vi "read-json-testing.vi"() -> ()   [LabVIEW 2019]
uses:
  <vilib>/Rock Robotics/WPI/ThirdParty/MJansen/PathPlanner/TypeDef/PathPlannerPath.ctl
  <vilib>/Rock Robotics/WPI/ThirdParty/MJansen/PathPlanner/TypeDef/PathPlannerRotationTarget.ctl
  <vilib>/Rock Robotics/WPI/ThirdParty/JAS_Junk/TrajLib/TypeDef/ROTATION2D.ctl
  <vilib>/Rock Robotics/WPI/ThirdParty/MJansen/PathPlanner/TypeDef/PathPlannerConstraintsZone.ctl
  <vilib>/Rock Robotics/WPI/ThirdParty/MJansen/PathPlanner/TypeDef/PathPlannerPathConstraints.ctl
  <vilib>/Rock Robotics/WPI/ThirdParty/MJansen/PathPlanner/TypeDef/PathPlannerEventMarker.ctl
  <vilib>/Rock Robotics/WPI/ThirdParty/MJansen/PathPlanner/TypeDef/PathPlannerCommandUtil.ctl
  <vilib>/Rock Robotics/WPI/ThirdParty/MJansen/PathPlanner/ENum/PathPlanner_CommandUtilType_ENUM.ctl
  <vilib>/Rock Robotics/WPI/ThirdParty/MJansen/PathPlanner/TypeDef/PathPlannerGoalEndState.ctl
  <vilib>/Rock Robotics/WPI/ThirdParty/MJansen/PathPlanner/TypeDef/PathPlannerPathPoint.ctl
  <vilib>/Rock Robotics/WPI/ThirdParty/JAS_Junk/TrajLib/TypeDef/TRANSLATION2D.ctl
  <vilib>/Rock Robotics/WPI/ThirdParty/MJansen/PathPlanner/TypeDef/PathPlannerWaypoint.ctl
  <vilib>/Rock Robotics/WPI/ThirdParty/MJansen/PathPlanner/TypeDef/PathPlannerPointTowardsZone.ctl
  <vilib>/Rock Robotics/WPI/ThirdParty/MJansen/PathPlanner/TypeDef/PathPlannerIdealStartingState.ctl
  <vilib>/Rock Robotics/WPI/ThirdParty/MJansen/PathPlanner/TypeDef/PathPlannerTrajectory.ctl
  <vilib>/Rock Robotics/WPI/ThirdParty/MJansen/PathPlanner/TypeDef/PathPlannerTrajectoryState.ctl
  <vilib>/Rock Robotics/WPI/ThirdParty/JAS_Junk/TrajLib/TypeDef/CHASSIS_SPEEDS.ctl
  <vilib>/Rock Robotics/WPI/ThirdParty/MJansen/PathPlanner/VI/PathPlanner_EventMarker_New.vi
  <vilib>/Rock Robotics/WPI/ThirdParty/MJansen/PathPlanner/VI/PathPlanner_CommandUtil_TypeFromString.vi
  <vilib>/Rock Robotics/WPI/ThirdParty/MJansen/PathPlanner/VI/PathPlanner_EventMarker_FromJSON_Data.vi
  <vilib>/Rock Robotics/WPI/ThirdParty/MJansen/PathPlanner/PathPlanner24.lvlib
  <vilib>/Rock Robotics/WPI/ThirdParty/JAS_Junk/TrajLib/Trajectory_Library.lvlib
panel:
  out "Exists":bool
  out "EventMarkers":T1[](array[typedef])
  in  "StartingSpeeds":T4 {"vOmega" format="%10.3f"; "vY" format="%10.3f"; "vX" format="%10.3f"}
  out "PathPlannerTrajectory":T5 {"States"."TargetHolonomicRotation"."SIN" format="%13.4f"; "States"."TargetHolonomicRotation"."COS" format="%13.4f"; "States"."TargetHolonomicRotation"."VALUE" format="%13.4f"; "States"."Heading"."SIN" format="%13.4f"; "States"."Heading"."COS" format="%13.4f"; "States"."Heading"."VALUE" format="%13.4f"; "States"."PositionMeters"."Y" format="%14.3f"; "States"."PositionMeters"."X" format="%14.3f"}
  out "Error":bool
  out "PathPlannerPath":T10={"Reversed"=FALSE, "RotationTargets"=[], "ConstraintZones"=[], "EventMarkers"=[], "GlobalConstraints"={"MaxVelocityMps;"=0.0, "MaxAccelerationMpsSq;"=0.0, "MaxAngularVelRadPsEc;"=0.0, "MaxAngularAccRadPSecSq"=0.0, "Exists"=FALSE, "Unlimited"=FALSE, "NominalVoltageVolts"=1.0}, "GoalEndState"={"VelocityMPS"=0.0, "Rotation"={"VALUE"=0.0, "COS"=1.0, "SIN"=0.0}}, "AllPoints"=[], "Name"="", "Waypoints"=[], "PointTowardsZones"=[], "IdealStartingState"={"VelocityMPS"=0.0, "Rotation"={"VALUE"=0.0, "COS"=1.0, "SIN"=0.0}}, "IsChoreoPath"=FALSE, "PreventFlipping"=FALSE} {"IdealStartingState"."Rotation"."SIN" format="%13.4f"; "IdealStartingState"."Rotation"."COS" format="%13.4f"; "IdealStartingState"."Rotation"."VALUE" format="%13.4f"; "PointTowardsZones"."TargetPosition"."Y" format="%14.3f"; "PointTowardsZones"."TargetPosition"."X" format="%14.3f"; "PointTowardsZones"."RotationOffset"."SIN" format="%13.4f"; "PointTowardsZones"."RotationOffset"."COS" format="%13.4f"; "PointTowardsZones"."RotationOffset"."VALUE" format="%13.4f"; "Waypoints"."nextControl"."Y" format="%14.3f"; "Waypoints"."nextControl"."X" format="%14.3f"; "Waypoints"."anchor"."Y" format="%14.3f"; "Waypoints"."anchor"."X" format="%14.3f"; "Waypoints"."prevControl"."Y" format="%14.3f"; "Waypoints"."prevControl"."X" format="%14.3f"; "AllPoints"."RotationTarget"."rotation"."SIN" format="%13.4f"; "AllPoints"."RotationTarget"."rotation"."COS" format="%13.4f"; "AllPoints"."RotationTarget"."rotation"."VALUE" format="%13.4f"; "AllPoints"."Position"."Y" format="%14.3f"; "AllPoints"."Position"."X" format="%14.3f"; "GoalEndState"."Rotation"."SIN" format="%13.4f"; "GoalEndState"."Rotation"."COS" format="%13.4f"; "GoalEndState"."Rotation"."VALUE" format="%13.4f"; "RotationTargets"."rotation"."SIN" format="%13.4f"; "RotationTargets"."rotation"."COS" format="%13.4f"; "RotationTargets"."rotation"."VALUE" format="%13.4f"}
  out "value 7":T18(array[cluster])
  out "error out 7":errorcluster
  in  "path 7":string[](array[string])=["rotationTargets"]
  in  "rotationTargets":T18(array[cluster])
  out "value 6":T19(array[cluster])
  out "error out 6":errorcluster
  in  "path 6":string[](array[string])=["eventMarkers"]
  in  "eventMarkers":T19(array[cluster])
  out "value 5":T20(array[cluster])
  out "error out 5":errorcluster
  in  "path 5":string[](array[string])=["constraintZones"]
  in  "constraintZones":T20(array[cluster])
  out "value 4":cluster{"velocity":dbl, "rotation":dbl}
  in  "goalEndstate":cluster{"velocity":dbl, "rotation":dbl}
  out "error out 4":errorcluster
  in  "path 4":string[](array[string])=["goalEndState"]
  out "value 3":bool
  out "error out 3":errorcluster
  in  "path 3":string[](array[string])=["reversed"]
  in  "reversed":bool
  out "value 2":T21
  out "error out 2":errorcluster
  in  "path 2":string[](array[string])=["globalConstraints"]
  in  "globalConstraints":T21
  out "value":T22(array[cluster])
  in  "waypoints":T22(array[cluster])
  in  "enable LabVIEW extensions? (T)":bool=TRUE
  in  "strict validation? (F)":bool
  in  "default null elements? (F)":bool=TRUE
  out "error out":errorcluster
  in  "path":string[](array[string])=["waypoints"]
  in  "json source":string="{\n  \"version\": \"2025.0\",\n  \"waypoints\": [\n    {\n      \"anchor\": {\n        \"x\": 2.0,\n        \"y\": 7.0\n      },\n      \"prevControl\": null,\n      \"nextControl\": {\n        \"x\": 3.58823932313598,\n        \"y\": 6.376881778529889\n      },\n      \"isLocked\": false,\n      \"linkedName\": null\n    },\n    {\n      \"anchor\": {\n        \"x\": 5.951268188250662,\n        \"y\": 5.597064479843246\n      },\n      \"prevControl\": {\n        \"x\": 4.577896893952,\n        \"y\": 6.542670794376735\n      },\n      \"nextControl\": {\n        \"x\": 6.508429267602249,\n        \"y\": 5.213442776787187\n      },\n      \"isLocked\": false,\n      \"linkedName\": null\n    },\n    {\n      \"anchor\": {\n        \"x\": 7.0,\n        \"y\": 1.0\n      },\n      \"prevControl\": {\n        \"x\": 6.6943943192889375,\n        \"y\": 1.9321390727468368\n      },\n      \"nextControl\": null,\n      \"isLocked\": false,\n      \"linkedName\": null\n    }\n  ],\n  \"rotationTargets\": [\n    {\n      \"waypointRelativePos\": 0.5,\n      \"rotationDegrees\": 0.0\n    }\n  ],\n  \"constraintZones\": [\n    {\n      \"name\": \"New Constraints Zone\",\n      \"minWaypointRelativePos\": 0.45,\n      \"maxWaypointRelativePos\": 0.7,\n      \"constraints\": {\n        \"maxVelocity\": 2.1,\n        \"maxAcceleration\": 2.2,\n        \"maxAngularVelocity\": 90.0,\n        \"maxAngularAcceleration\": 91.0,\n        \"nominalVoltage\": 12.0,\n        \"unlimited\": false\n      }\n    }\n  ],\n  \"pointTowardsZones\": [\n    {\n      \"fieldPosition\": {\n        \"x\": 6.0,\n        \"y\": 5.5\n      },\n      \"rotationOffset\": -20.0,\n      \"minWaypointRelativePos\": 0.4952380952380946,\n      \"maxWaypointRelativePos\": 1.0047619047619045,\n      \"name\": \"Point Towards Zone\"\n    }\n  ],\n  \"eventMarkers\": [\n    {\n      \"name\": \"event-1\",\n      \"waypointRelativePos\": 0.35,\n      \"endWaypointRelativePos\": null,\n      \"command\": {\n        \"type\": \"parallel\",\n        \"data\": {\n          \"commands\": [\n            {\n              \"type\": \"named\",\n              \"data\": {\n                \"name\": \"jim1\"\n              }\n            },\n            {\n              \"type\": \"named\",\n              \"data\": {\n                \"name\": \"jim2\"\n              }\n            }\n          ]\n        }\n      }\n    },\n    {\n      \"name\": \"event-2\",\n      \"waypointRelativePos\": 0.85,\n      \"endWaypointRelativePos\": null,\n      \"command\": {\n        \"type\": \"sequential\",\n        \"data\": {\n          \"commands\": [\n            {\n              \"type\": \"named\",\n              \"data\": {\n                \"name\": \"jim3\"\n              }\n            },\n            {\n              \"type\": \"wait\",\n              \"data\": {\n                \"waitTime\": 0.24\n              }\n            }\n          ]\n        }\n      }\n    },\n    {\n      \"name\": \"event-3\",\n      \"waypointRelativePos\": 1.3,\n      \"endWaypointRelativePos\": null,\n      \"command\": {\n        \"type\": \"deadline\",\n        \"data\": {\n          \"commands\": [\n            {\n              \"type\": \"named\",\n              \"data\": {\n                \"name\": \"jim4\"\n              }\n            }\n          ]\n        }\n      }\n    },\n    {\n      \"name\": \"event-4\",\n      \"waypointRelativePos\": 1.85,\n      \"endWaypointRelativePos\": null,\n      \"command\": {\n        \"type\": \"race\",\n        \"data\": {\n          \"commands\": [\n            {\n              \"type\": \"sequential\",\n              \"data\": {\n                \"commands\": [\n                  {\n                    \"type\": \"wait\",\n                    \"data\": {\n                      \"waitTime\": 0.1\n                    }\n                  },\n                  {\n                    \"type\": \"named\",\n                    \"data\": {\n                      \"name\": \"jim5\"\n                    }\n                  }\n                ]\n              }\n            }\n          ]\n        }\n      }\n    }\n  ],\n  \"globalConstraints\": {\n    \"maxVelocity\": 3.0,\n    \"maxAcceleration\": 3.0,\n    \"maxAngularVelocity\": 540.0,\n    \"maxAngularAcceleration\": 720.0,\n    \"nominalVoltage\": 12.0,\n    \"unlimited\": false\n  },\n  \"goalEndState\": {\n    \"velocity\": 0.0,\n    \"rotation\": -75.0\n  },\n  \"reversed\": false,\n  \"folder\": null,\n  \"idealStartingState\": {\n    \"velocity\": 0,\n    \"rotation\": 20.0\n  },\n  \"useDefaultConstraints\": false\n}"
  # "Not an issue.   The real VI\nworks correctly!"
  # "\"rotationTargets\": [\n    {\n      \"waypointRelativePos\": 0.5,\n      \"rotationDegrees\": 0.0\n    }\n  ],"
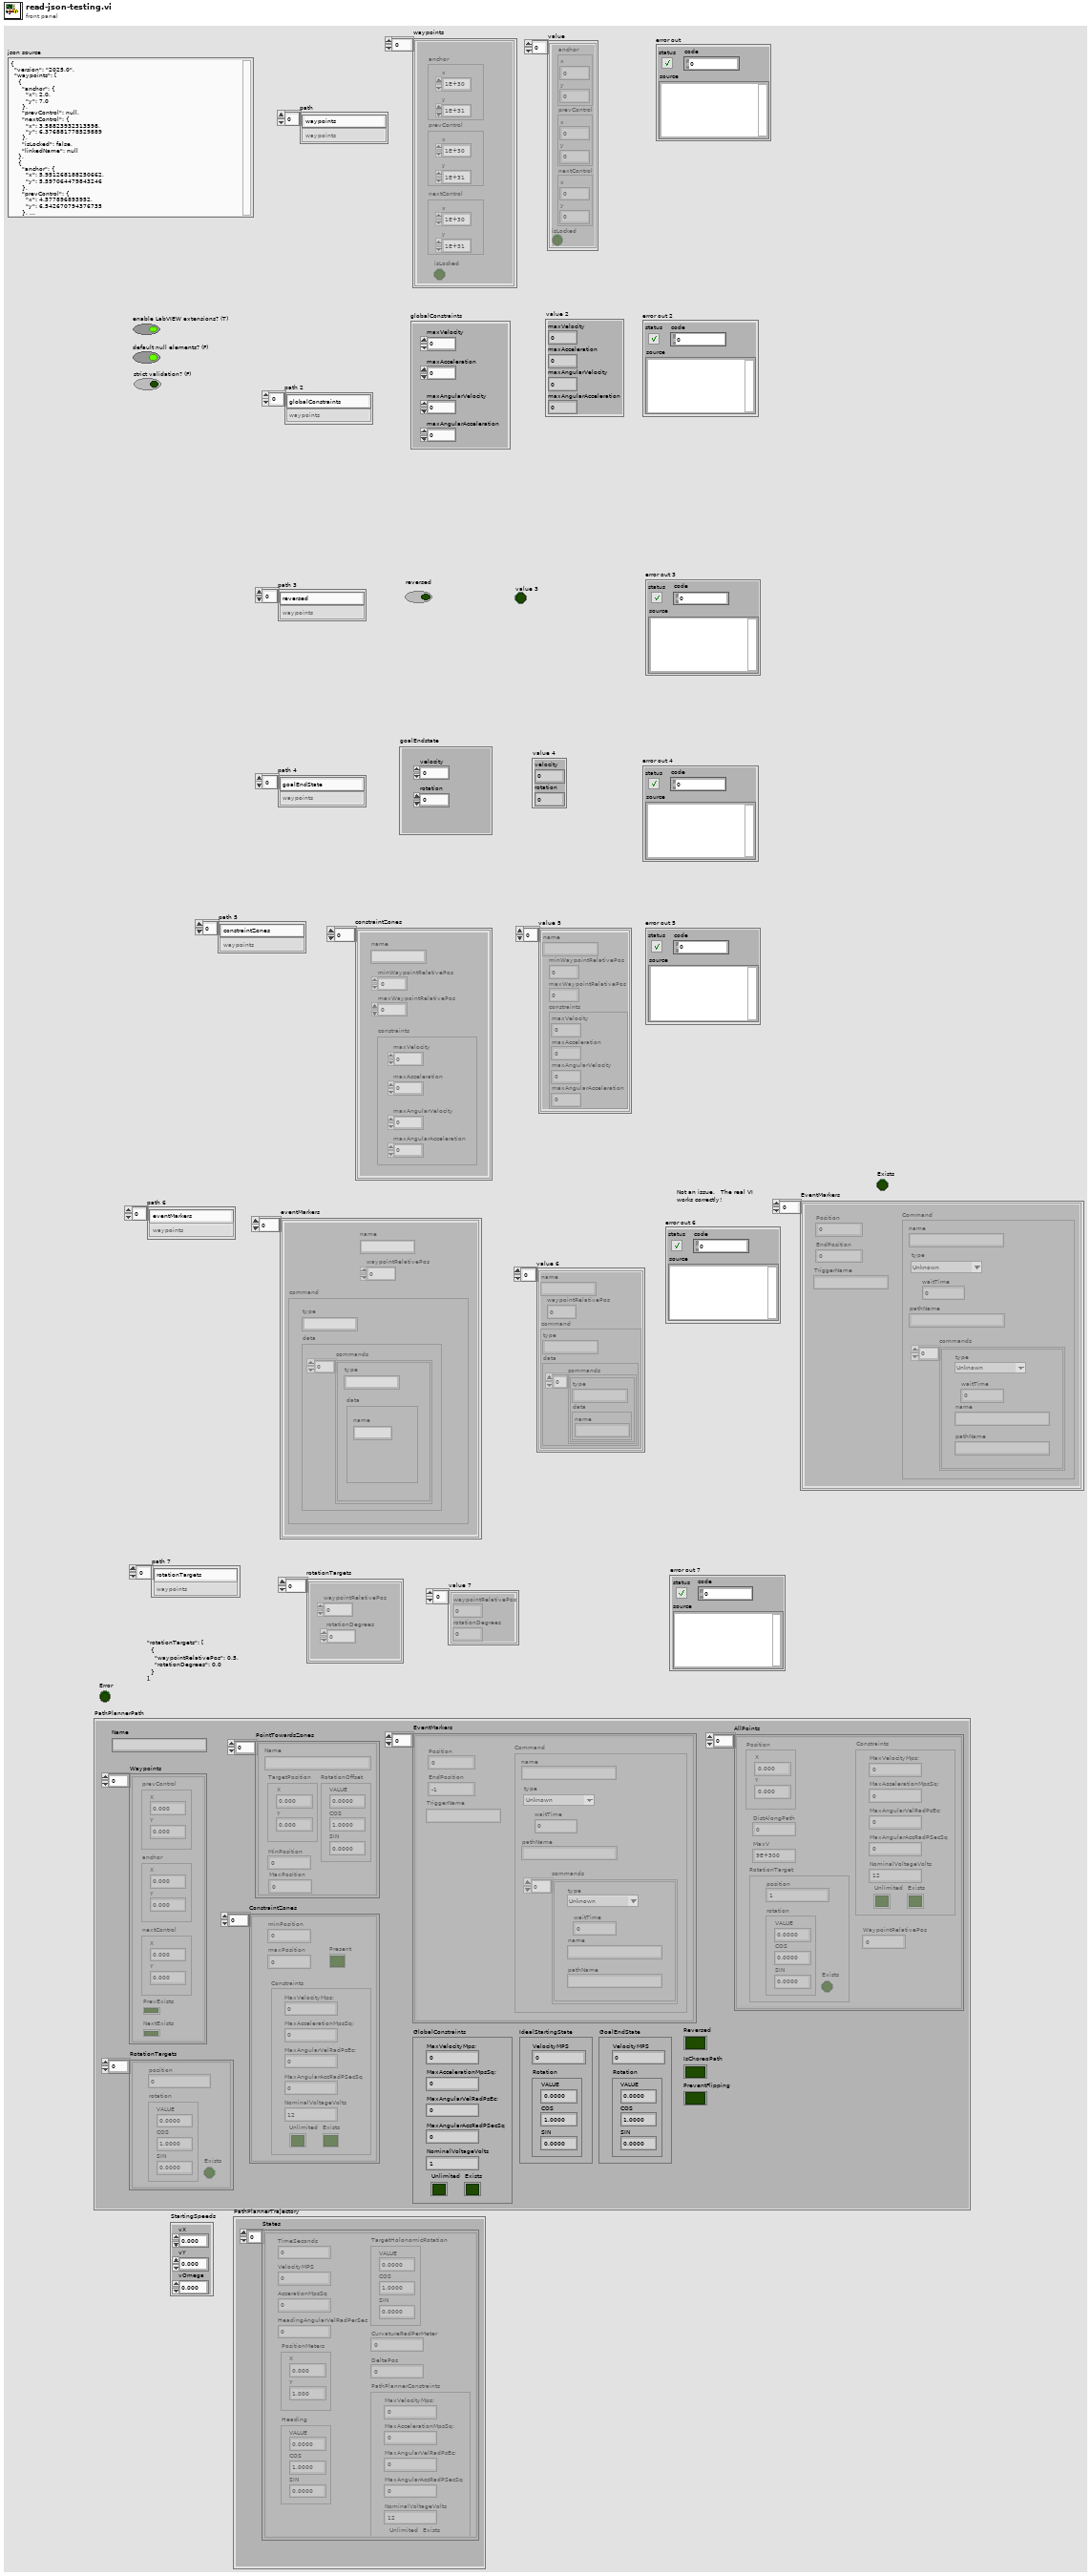
[diagram p1: front panel]
types:
  T1 = typedef "PathPlanner24.lvlib/PathPlannerEventMarker.ctl" = cluster{"Position":dbl, "Command":T2, "TriggerName":string, "EndPosition":dbl}
  T2 = typedef "PathPlanner24.lvlib/PathPlannerCommandUtil.ctl" = cluster{"waitTime":dbl, "name":string, "pathName":string, "commands":cluster{"type":T3, "waitTime":dbl, "name":string, "pathName":string}[], "type":T3}
  T3 = typedef "PathPlanner24.lvlib/PathPlanner_CommandUtilType_ENUM.ctl" = enum16{"Unknown", "Wait", "Named", "Path", "Sequential", "Parallel", "Race", "Deadline"}
  T4 = typedef "Trajectory_Library.lvlib/CHASSIS_SPEEDS.ctl" = cluster{"vX":dbl, "vY":dbl, "vOmega":dbl}
  T5 = typedef "PathPlanner24.lvlib/PathPlannerTrajectory.ctl" = cluster{"States":T6[]}
  T6 = typedef "PathPlanner24.lvlib/PathPlannerTrajectoryState.ctl" = cluster{"TimeSeconds":dbl, "VelocityMPS":dbl, "AccerationMpsSq":dbl, "HeadingAngularVelRadPerSec":dbl, "PositionMeters":T7, "Heading":T8, "TargetHolonomicRotation":T8, "CurvatureRadPerMeter":dbl, "PathPlannerConstraints":T9, "DeltaPos":dbl}
  T7 = typedef "Trajectory_Library.lvlib/TRANSLATION2D.ctl" = cluster{"X":dbl, "Y":dbl}
  T8 = typedef "Trajectory_Library.lvlib/ROTATION2D.ctl" = cluster{"VALUE":dbl, "COS":dbl, "SIN":dbl}
  T9 = typedef "PathPlanner24.lvlib/PathPlannerPathConstraints.ctl" = cluster{"MaxVelocityMps;":dbl, "MaxAccelerationMpsSq;":dbl, "MaxAngularVelRadPsEc;":dbl, "MaxAngularAccRadPSecSq":dbl, "Exists":bool, "Unlimited":bool, "NominalVoltageVolts":dbl}
  T10 = typedef "PathPlanner24.lvlib/PathPlannerPath.ctl" = cluster{"Reversed":bool, "RotationTargets":T11[], "ConstraintZones":T12[], "EventMarkers":T1[], "GlobalConstraints":T9, "GoalEndState":T13, "AllPoints":T14[], "Name":string, "Waypoints":T15[], "PointTowardsZones":T16[], "IdealStartingState":T17, "IsChoreoPath":bool, "PreventFlipping":bool}
  T11 = typedef "PathPlanner24.lvlib/PathPlannerRotationTarget.ctl" = cluster{"position":dbl, "rotation":T8, "Exists":bool}
  T12 = typedef "PathPlanner24.lvlib/PathPlannerConstraintsZone.ctl" = cluster{"minPosition":dbl, "maxPosition":dbl, "Constraints":T9, "Present":bool}
  T13 = typedef "PathPlanner24.lvlib/PathPlannerGoalEndState.ctl" = cluster{"VelocityMPS":dbl, "Rotation":T8}
  T14 = typedef "PathPlanner24.lvlib/PathPlannerPathPoint.ctl" = cluster{"Position":T7, "DistAlongPath":dbl, "MaxV":dbl, "Constraints":T9, "RotationTarget":T11, "WaypointRelativePos":dbl}
  T15 = typedef "PathPlanner24.lvlib/PathPlannerWaypoint.ctl" = cluster{"prevControl":T7, "anchor":T7, "nextControl":T7, "PrevExists":bool, "NextExists":bool}
  T16 = typedef "PathPlanner24.lvlib/PathPlannerPointTowardsZone.ctl" = cluster{"RotationOffset":T8, "Name":string, "TargetPosition":T7, "MinPosition":dbl, "MaxPosition":dbl}
  T17 = typedef "PathPlanner24.lvlib/PathPlannerIdealStartingState.ctl" = cluster{"VelocityMPS":dbl, "Rotation":T8}
  T18 = cluster{"waypointRelativePos":dbl, "rotationDegrees":dbl}[]
  T19 = cluster{"name":string, "waypointRelativePos":dbl, "command":cluster{"type":string, "data":cluster{"commands":cluster{"type":string, "data":cluster{"name":string}}[]}}}[]
  T20 = cluster{"name":string, "minWaypointRelativePos":dbl, "maxWaypointRelativePos":dbl, "constraints":cluster{"maxVelocity":dbl, "maxAcceleration":dbl, "maxAngularVelocity":dbl, "maxAngularAcceleration":dbl}}[]
  T21 = cluster{"maxVelocity":dbl, "maxAcceleration":dbl, "maxAngularVelocity":dbl, "maxAngularAcceleration":dbl}
  T22 = cluster{"anchor":cluster{"x":dbl, "y":dbl}, "prevControl":cluster{"x":dbl, "y":dbl}, "nextControl":cluster{"x":dbl, "y":dbl}, "isLocked":bool}[]
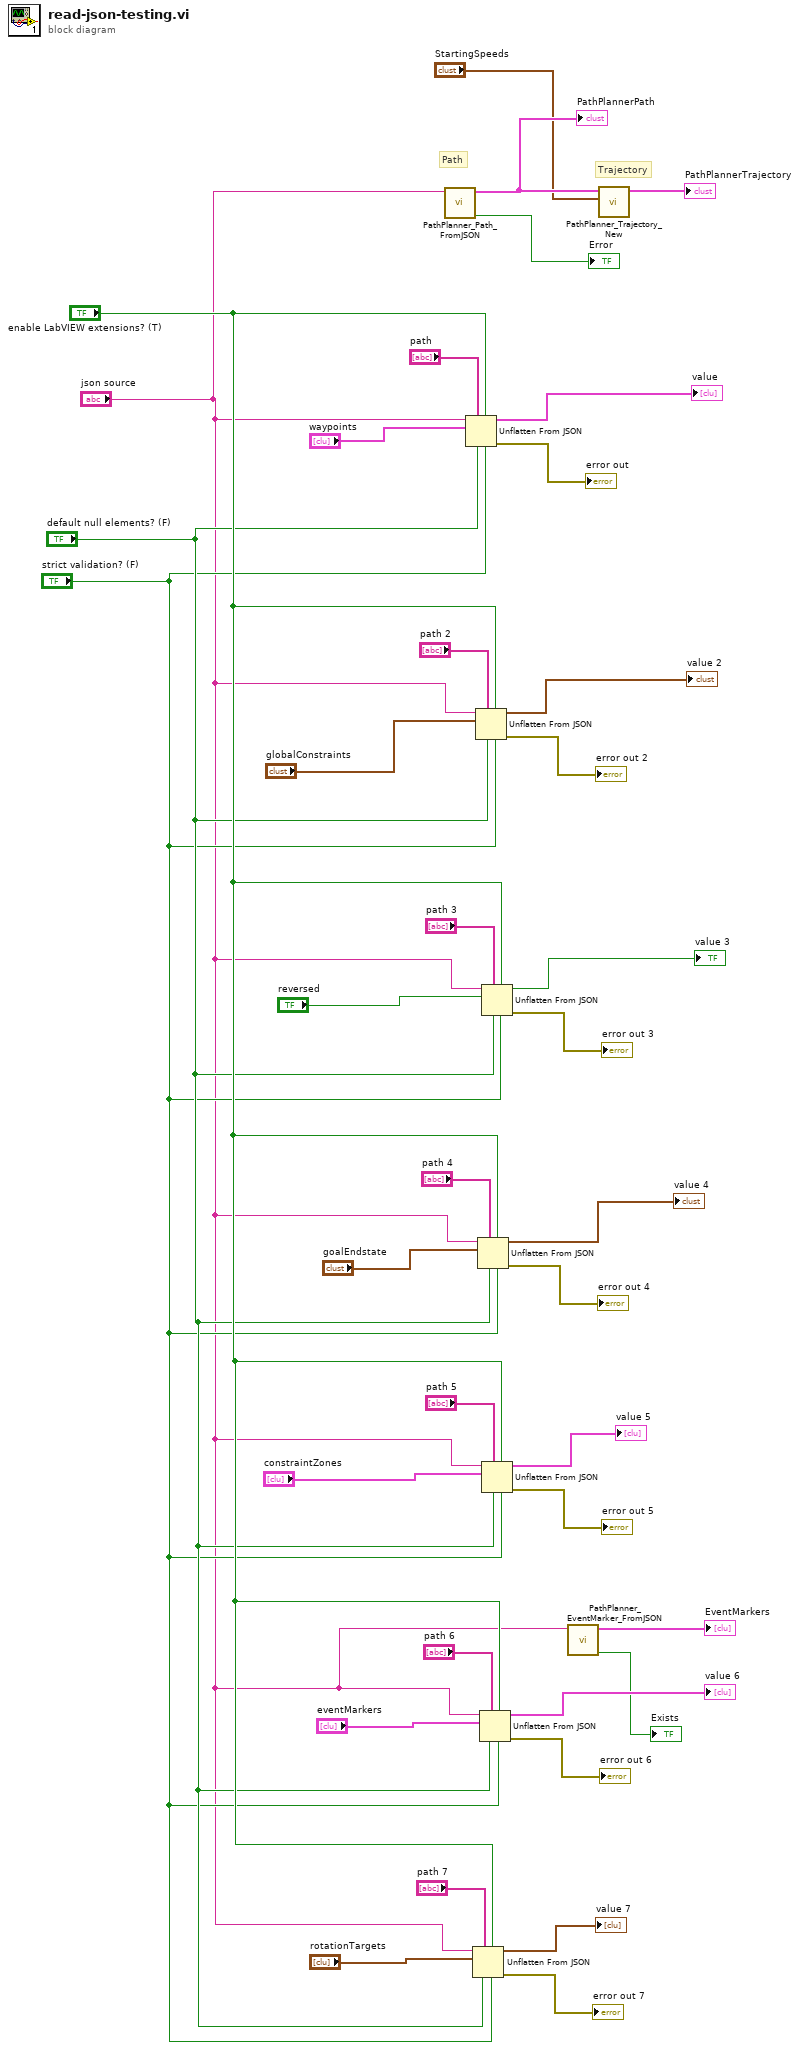
[diagram p0: block diagram]
diagram:
  # "Trajectory"
  # "Path"
  n1 = call <vilib>:"PathPlanner_Path_FromJSON.vi"("JSON String"="json source") -> ("Error"=→"Error":bool, "PathPlannerPath"=w6:T10)  [unwired: 8 in, 1 out]
  "PathPlannerPath" <- w6
  n2 = Unflatten From JSON(path="path", enable LabVIEW extensions? (T)="enable LabVIEW extensions? (T)", JSON string="json source", type and defaults="waypoints", default null elements? (F)="default null elements? (F)", strict validation? (F)="strict validation? (F)") -> (value=→"value":T22, error out=→"error out":errorcluster)  [unwired: 1 in]
  n3 = Unflatten From JSON(path="path 7", enable LabVIEW extensions? (T)="enable LabVIEW extensions? (T)", JSON string="json source", type and defaults="rotationTargets", default null elements? (F)="default null elements? (F)", strict validation? (F)="strict validation? (F)") -> (value=→"value 7":T18, error out=→"error out 7":errorcluster)  [unwired: 1 in]
  n4 = Unflatten From JSON(path="path 2", enable LabVIEW extensions? (T)="enable LabVIEW extensions? (T)", JSON string="json source", type and defaults="globalConstraints", default null elements? (F)="default null elements? (F)", strict validation? (F)="strict validation? (F)") -> (value=→"value 2":T21, error out=→"error out 2":errorcluster)  [unwired: 1 in]
  n5 = Unflatten From JSON(path="path 4", enable LabVIEW extensions? (T)="enable LabVIEW extensions? (T)", JSON string="json source", type and defaults="goalEndstate", default null elements? (F)="default null elements? (F)", strict validation? (F)="strict validation? (F)") -> (value=→"value 4":cluster{"velocity":dbl, "rotation":dbl}, error out=→"error out 4":errorcluster)  [unwired: 1 in]
  n6 = Unflatten From JSON(path="path 6", enable LabVIEW extensions? (T)="enable LabVIEW extensions? (T)", JSON string="json source", type and defaults="eventMarkers", default null elements? (F)="default null elements? (F)", strict validation? (F)="strict validation? (F)") -> (value=→"value 6":T19, error out=→"error out 6":errorcluster)  [unwired: 1 in]
  n7 = Unflatten From JSON(path="path 3", enable LabVIEW extensions? (T)="enable LabVIEW extensions? (T)", JSON string="json source", type and defaults="reversed", default null elements? (F)="default null elements? (F)", strict validation? (F)="strict validation? (F)") -> (value=→"value 3":bool, error out=→"error out 3":errorcluster)  [unwired: 1 in]
  n8 = Unflatten From JSON(path="path 5", enable LabVIEW extensions? (T)="enable LabVIEW extensions? (T)", JSON string="json source", type and defaults="constraintZones", default null elements? (F)="default null elements? (F)", strict validation? (F)="strict validation? (F)") -> (value=→"value 5":T20, error out=→"error out 5":errorcluster)  [unwired: 1 in]
  n9 = call <vilib>:"PathPlanner_EventMarker_FromJSON.vi"("JSON String"="json source") -> ("Exists"=→"Exists":bool, "EventMarkers"=→"EventMarkers":T1[])  [unwired: 9 in]
  n10 = call <vilib>:"PathPlanner_Trajectory_New.vi"("StartingSpeeds"="StartingSpeeds", "Path"=w6) -> ("PathPlannerTrajectory"=→"PathPlannerTrajectory":T5)  [unwired: 8 in, 1 out]
